vi "UI Updater Events.vi"() -> (0 "UI Updater":T1)   [LabVIEW 2018, in "GLog.lvlib" / "UI Updater.lvlib"]
uses:
  UI Updater.lvlib
  Events.ctl
  Write Log.ctl
  Register.ctl
  Unregister.ctl
  Unregister Response Data.ctl
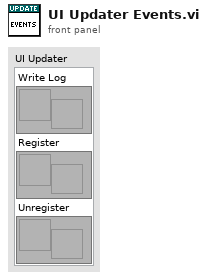
[diagram p1: front panel]
types:
  T1 = typedef "GLog.lvlib/UI Updater.lvlib/Events.ctl" = cluster{"Write Log":refnum<user-event>, "Register":refnum<user-event>, "Unregister":refnum<user-event>}
  T2 = typedef "GLog.lvlib/UI Updater.lvlib/Write Log.ctl" = cluster{"handler name":string, "formatted record":string}
  T3 = typedef "GLog.lvlib/UI Updater.lvlib/Register.ctl" = cluster{"Handler Name":string, "Ctl Ref":refnum<vi>, "Log Limit":i32, "Line Limit":i32, "AutoScroll?":bool}
  T4 = typedef "GLog.lvlib/UI Updater.lvlib/Unregister.ctl" = cluster{"handler name":string, "response notifier":refnum<notifier>}
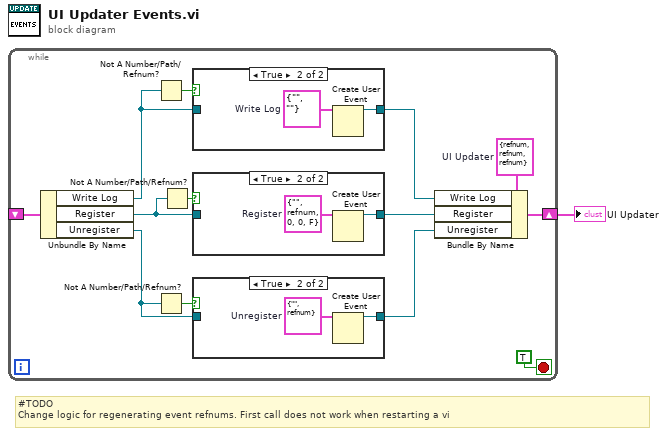
[diagram p0: block diagram]
diagram:
  # "#TODO\nChange logic for regenerating event refnums. First call does not work when restarting a vi"
  n1 = while {
    shift-right: [w14] -> w1
    shift-left: _ -> [w9]
    stop <- TRUE stop-if-true
    w2 = T1 {"Write Log"=refnum, "Register"=refnum, "Unregister"=refnum}  # UI Updater
    n2 = Unbundle By Name(w9) -> ("Write Log"=w3:refnum<user-event>, "Register"=w5:refnum<user-event>, "Unregister"=w4:refnum<user-event>)
    n3 = Not A Number/Path/Refnum?(number/path/refnum=w3) -> (NaN/Path/Refnum?=w8:bool)
    n4 = Not A Number/Path/Refnum?(number/path/refnum=w4) -> (NaN/Path/Refnum?=w7:bool)
    n5 = Not A Number/Path/Refnum?(number/path/refnum=w5) -> (NaN/Path/Refnum?=w6:bool)
    n6 = case shown="True" w8 {
      tunnel: [w21 w23] -> w12
      tunnel: w3 -> [w21 _]
      frame False {
      }
      frame True {
        w22 = T2 {"handler name"="", "formatted record"=""}  # Write Log
        n7 = Create User Event(user event datatype=w22) -> (user event=w23:refnum<user-event>)  [unwired: 1 in, 1 out]
      }
    }
    n8 = case shown="True" w6 {
      tunnel: [w18 w20] -> w10
      tunnel: w5 -> [w18 _]
      frame False {
      }
      frame True {
        w19 = T3 {"Handler Name"="", "Ctl Ref"=refnum, "Log Limit"=0, "Line Limit"=0, "AutoScroll?"=FALSE}  # Register
        n9 = Create User Event(user event datatype=w19) -> (user event=w20:refnum<user-event>)  [unwired: 1 in, 1 out]
      }
    }
    n10 = case shown="True" w7 {
      tunnel: [w15 w17] -> w11
      tunnel: w4 -> [w15 _]
      frame False {
      }
      frame True {
        w16 = T4 {"handler name"="", "response notifier"=refnum}  # Unregister
        n11 = Create User Event(user event datatype=w16) -> (user event=w17:refnum<user-event>)  [unwired: 1 in, 1 out]
      }
    }
    n12 = Bundle By Name(cluster=w2, "Write Log"=w12, "Register"=w10, "Unregister"=w11) -> (w14:T1)
  }
  "UI Updater" <- w1
